vi "PicoReadPicoSingleBuffers.vi"(1 "enabled array":i16[](array[numeric]), 2 "Buffer and Transfer Settings":T3={"startIndex"=0, "Samples"=1000000, "Down Sample Ratio"=1, "Down-Sample Mode"=2147483648} {"Down-Sample Mode" items=["RAW none"=2147483648, "None"=0, "Aggregate"=1, "Decimate"=2, "Average"=4]; "Down Sample Ratio" step=1; "Samples" format="%_6p"}, 3 "Variant":string, 5 "Data Pointers":T2, 9 "Buffer Number":i32=1, 11 "error in (no error)":errorcluster) -> (6 "MaxBuffers (Max or non-aggregated)":T1, 8 "Min Buffers":T1, 15 "error out":errorcluster)   [LabVIEW 2010]
doc: "Read data from a single Picodata buffer."
uses:
  PicoBuffers.ctl
  Buffer and Transfer Settings.ctl
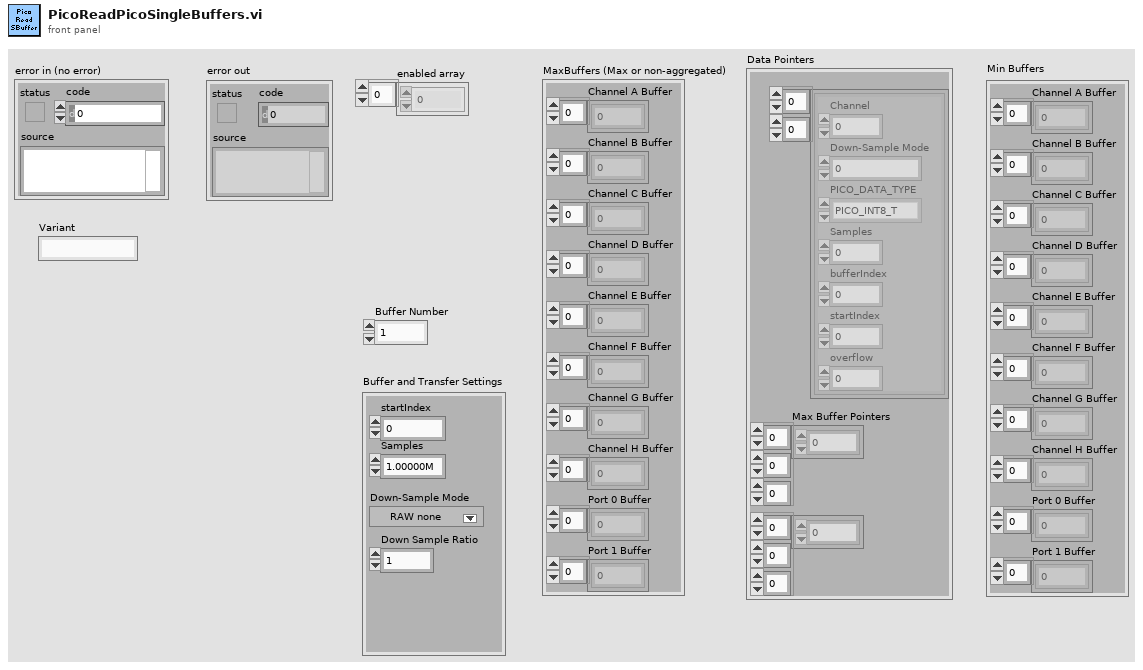
[diagram p1: front panel]
types:
  T1 = cluster{"Channel A Buffer":i16[], "Channel B Buffer":i16[], "Channel C Buffer":i16[], "Channel D Buffer":i16[], "Channel E Buffer":i16[], "Channel F Buffer":i16[], "Channel G Buffer":i16[], "Channel H Buffer":i16[], "Port 0 Buffer":i16[], "Port 1 Buffer":i16[]}
  T2 = typedef "PicoBuffers.ctl" = cluster{"Max Buffer Pointers":u64[][][], "Min Buffer Pointers":u64[][][], "StreamingDataInfo":cluster{"Channel":u32, "Down-Sample Mode":u32, "PICO_DATA_TYPE":enum32{"PICO_INT8_T", "PICO_INT16_T", "PICO_INT32_T", "PICO_UINT32_T", "PICO_INT64_T", ""}, "Samples":i32, "bufferIndex":u64, "startIndex":i32, "overflow":i16}[][]}
  T3 = typedef "Buffer and Transfer Settings.ctl" = cluster{"startIndex":u64, "Samples":u64, "Down Sample Ratio":u64, "Down-Sample Mode":u32}
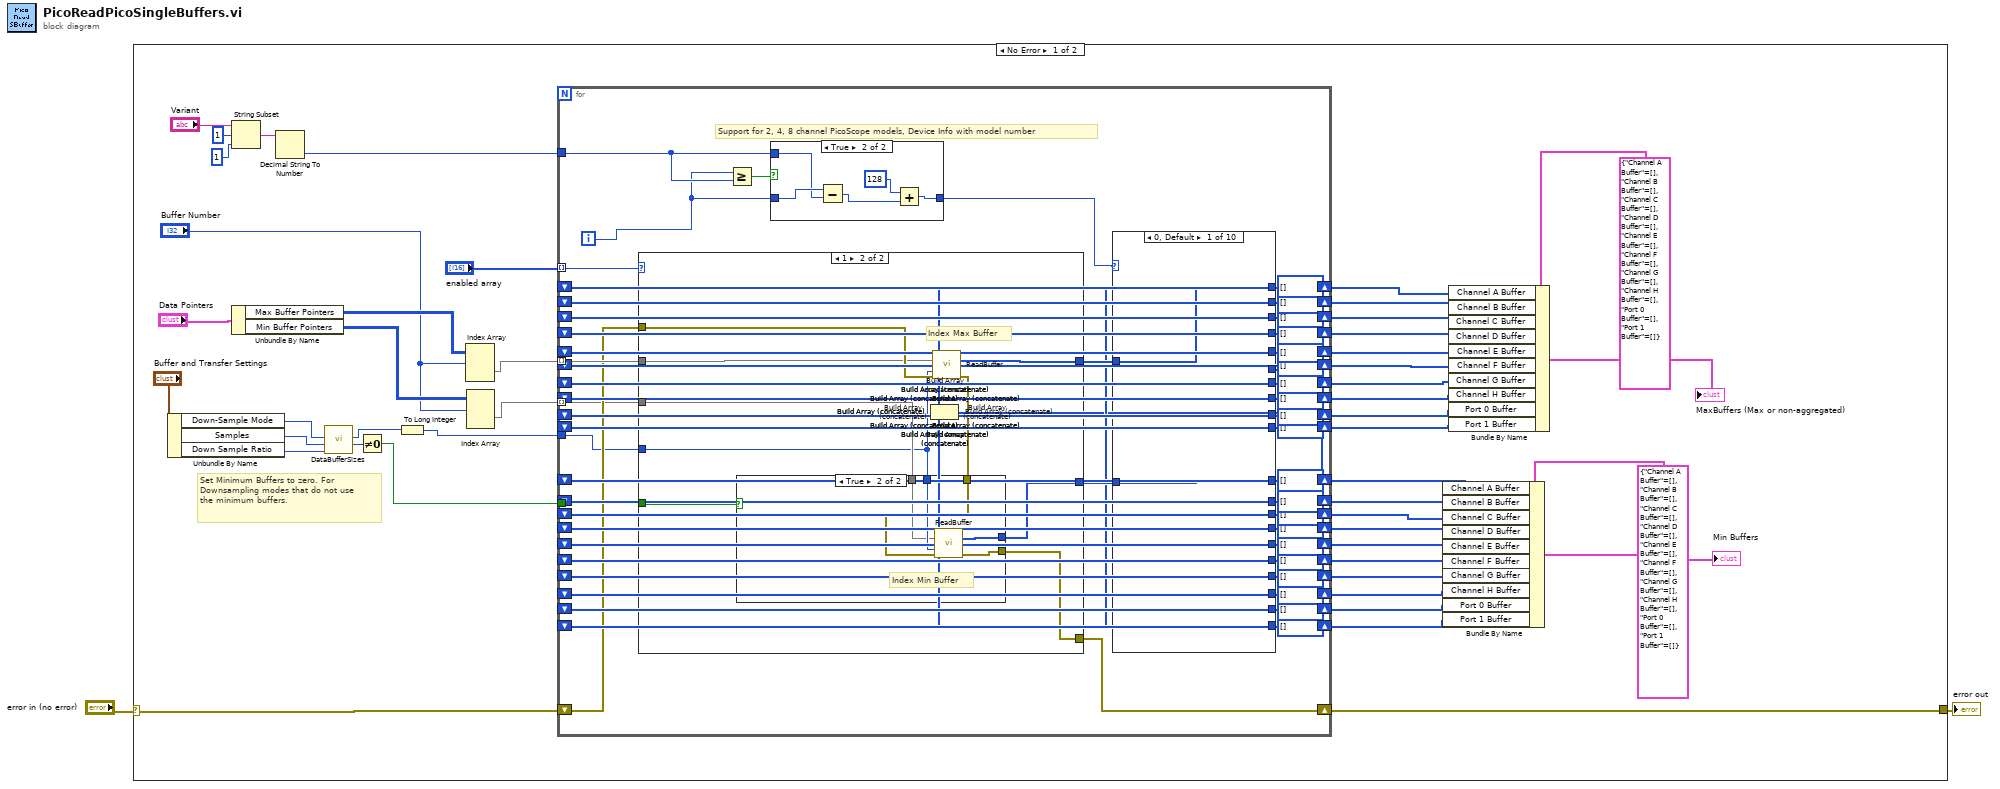
[diagram p0: block diagram]
diagram:
  n1 = case shown="No Error" "error in (no error)" {
    selector: "error in (no error)" -> [w66 w184]
    tunnel: [w68 w184] -> w1
    frame No Error {
      # "Set Minimum Buffers to zero. For Downsampling modes that do not use the minimum buffers."
      n2 = Unbundle By Name("Buffer and Transfer Settings") -> ("Down-Sample Mode"=w64:u32, "Samples"=w63:u64, "Down Sample Ratio"=w65:u64)
      n3 = Unbundle By Name("Data Pointers") -> ("Max Buffer Pointers"=w29:u64[][][], "Min Buffer Pointers"=w28:u64[][][])
      n4 = String Subset(string="Variant", offset (0)=1, length (rest)=1 ("length (rest)")) -> (substring=w57:string)
      n5 = Decimal String To Number(string=w57) -> (number=w23:i32)  [unwired: 2 in, 1 out]
      n6 = call "DataBufferSizes.vi"("Down Sample Ratio"=w65, "Number of Samples"=w63, "Down-Sample Mode"=w64) -> ("min Buffer Size"=w61:i32, "Max Buffer Size"=w59:i32)  [unwired: 7 in]
      n7 = Not Equal To 0?(x=w61) -> (x != 0?=w62:bool)
      n8 = To Long Integer(number=w59) -> (32bit integer=w60:i32)
      n9 = Index Array(array=w29, index (dim 0)="Buffer Number") -> (element=w27:u64[][])  [unwired: 2 in]
      n10 = Index Array(array=w28, index (dim 0)="Buffer Number") -> (element=w26:u64[][])  [unwired: 2 in]
      n11 = for {
        tunnel: "enabled array" -> [w140] mode=indexing
        tunnel: w27 -> [w141] mode=indexing
        shift-right: [w139] -> w68
        shift-left: w66 -> [w138]
        tunnel: w60 -> [w124]
        tunnel: w62 -> [w123]
        tunnel: w26 -> [w113] mode=indexing
        tunnel: w23 -> [w110]
        shift-right: [w107] -> w53
        shift-left: i16[] [] ("Output Array") -> [w108]
        shift-right: [w105] -> w52
        shift-left: i16[] [] ("Output Array") -> [w106]
        shift-right: [w103] -> w51
        shift-left: i16[] [] ("Output Array") -> [w104]
        shift-right: [w101] -> w50
        shift-left: i16[] [] ("Output Array") -> [w102]
        shift-right: [w99] -> w49
        shift-left: i16[] [] ("Output Array") -> [w100]
        shift-right: [w97] -> w48
        shift-left: i16[] [] ("Output Array") -> [w98]
        shift-right: [w95] -> w42
        shift-left: i16[] [] ("Output Array") -> [w96]
        shift-right: [w93] -> w47
        shift-left: i16[] [] ("Output Array") -> [w94]
        shift-right: [w91] -> w46
        shift-left: i16[] [] ("Output Array") -> [w92]
        shift-right: [w89] -> w45
        shift-left: i16[] [] ("Output Array") -> [w90]
        shift-right: [w87] -> w44
        shift-left: i16[] [] ("Output Array") -> [w88]
        shift-right: [w85] -> w43
        shift-left: i16[] [] ("Output Array") -> [w86]
        shift-right: [w83] -> w39
        shift-left: i16[] [] ("Output Array") -> [w84]
        shift-right: [w81] -> w38
        shift-left: i16[] [] ("Output Array") -> [w82]
        shift-right: [w79] -> w37
        shift-left: i16[] [] ("Output Array") -> [w80]
        shift-right: [w77] -> w36
        shift-left: i16[] [] ("Output Array") -> [w78]
        shift-right: [w75] -> w35
        shift-left: i16[] [] ("Output Array") -> [w76]
        shift-right: [w73] -> w34
        shift-left: i16[] [] ("Output Array") -> [w74]
        shift-right: [w71] -> w33
        shift-left: i16[] [] ("Output Array") -> [w72]
        shift-right: [w69] -> w32
        shift-left: i16[] [] ("Output Array") -> [w70]
        i -> [w109]
        # "Support for 2, 4, 8 channel PicoScope models, Device Info with model number"
        n12 = case shown="1" w140 {
          tunnel: w141 -> [_ w171]
          tunnel: [_ w177] -> w137
          tunnel: [_ w176] -> w136
          tunnel: w138 -> [w168 w175]
          tunnel: [w168 w173] -> w139
          tunnel: w124 -> [_ w169]
          tunnel: w123 -> [_ w172]
          tunnel: w113 -> [_ w170]
          frame 0, Default {
          }
          frame 1 {
            # "Index Max Buffer"
            n13 = call "ReadBuffer.vi"("Pointer and BufferSize"=w171, "Buffer size"=w169, "error in (no error)"=w175) -> ("Output Array"=w177:i16[], "error out"=w174:errorcluster)  [unwired: 11 in]
            n14 = case shown="True" w172 {
              tunnel: [_ w183] -> w176
              tunnel: w174 -> [w178 w182]
              tunnel: [w178 w181] -> w173
              tunnel: w169 -> [_ w180]
              tunnel: w170 -> [_ w179]
              frame False {
              }
              frame True {
                # "Index Min Buffer"
                n15 = call "ReadBuffer.vi"("Pointer and BufferSize"=w179, "Buffer size"=w180, "error in (no error)"=w182) -> ("Output Array"=w183:i16[], "error out"=w181:errorcluster)  [unwired: 11 in]
              }
            }
          }
        }
        n16 = Greater Or Equal?(x=w109, y=w110) -> (x >= y?=w112:bool)
        n17 = case shown="True" w112 {
          tunnel: w109 -> [w142 w144]
          tunnel: [w142 w146] -> w111
          tunnel: w110 -> [_ w143]
          frame False {
          }
          frame True {
            n18 = Subtract(x=w144, y=w143) -> (x-y=w145:i32)
            n19 = Add(x=128, y=w145) -> (x+y=w146:i32)
          }
        }
        n20 = case shown="0, Default" w111 {
          tunnel: w137 -> [w149 w151 w153 w155 w157 w159 w161 w163 w165 w167]
          tunnel: [w149 _ _ _ _ _ _ _ _ _] -> w122
          tunnel: [_ w151 _ _ _ _ _ _ _ _] -> w129
          tunnel: [_ _ w153 _ _ _ _ _ _ _] -> w128
          tunnel: [_ _ _ w155 _ _ _ _ _ _] -> w127
          tunnel: [_ _ _ _ w157 _ _ _ _ _] -> w126
          tunnel: [_ _ _ _ _ w159 _ _ _ _] -> w125
          tunnel: w136 -> [w148 w150 w152 w154 w156 w158 w160 w162 w164 w166]
          tunnel: [w148 _ _ _ _ _ _ _ _ _] -> w135
          tunnel: [_ w150 _ _ _ _ _ _ _ _] -> w134
          tunnel: [_ _ w152 _ _ _ _ _ _ _] -> w133
          tunnel: [_ _ _ w154 _ _ _ _ _ _] -> w132
          tunnel: [_ _ _ _ w156 _ _ _ _ _] -> w131
          tunnel: [_ _ _ _ _ w158 _ _ _ _] -> w130
          tunnel: [_ _ _ _ _ _ w161 _ _ _] -> w121
          tunnel: [_ _ _ _ _ _ w160 _ _ _] -> w120
          tunnel: [_ _ _ _ _ _ _ w163 _ _] -> w119
          tunnel: [_ _ _ _ _ _ _ w162 _ _] -> w118
          tunnel: [_ _ _ _ _ _ _ _ w165 _] -> w117
          tunnel: [_ _ _ _ _ _ _ _ w164 _] -> w116
          tunnel: [_ _ _ _ _ _ _ _ _ w167] -> w115
          tunnel: [_ _ _ _ _ _ _ _ _ w166] -> w114
          frame 0, Default {
          }
          frame 1 {
          }
          frame 2 {
          }
          frame 3 {
          }
          frame 4 {
          }
          frame 5 {
          }
          frame 6 {
          }
          frame 7 {
          }
          frame 128 {
          }
          frame 129 {
          }
        }
        n21 = Build Array (concatenate)(w70, w114) -> (w69:i16[])
        n22 = Build Array (concatenate)(w72, w115) -> (w71:i16[])
        n23 = Build Array (concatenate)(w74, w116) -> (w73:i16[])
        n24 = Build Array (concatenate)(w76, w117) -> (w75:i16[])
        n25 = Build Array (concatenate)(w78, w118) -> (w77:i16[])
        n26 = Build Array (concatenate)(w80, w119) -> (w79:i16[])
        n27 = Build Array (concatenate)(w82, w120) -> (w81:i16[])
        n28 = Build Array (concatenate)(w84, w121) -> (w83:i16[])
        n29 = Build Array (concatenate)(w86, w125) -> (w85:i16[])
        n30 = Build Array (concatenate)(w88, w126) -> (w87:i16[])
        n31 = Build Array (concatenate)(w90, w127) -> (w89:i16[])
        n32 = Build Array (concatenate)(w92, w128) -> (w91:i16[])
        n33 = Build Array (concatenate)(w94, w129) -> (w93:i16[])
        n34 = Build Array (concatenate)(w96, w122) -> (w95:i16[])
        n35 = Build Array (concatenate)(w98, w130) -> (w97:i16[])
        n36 = Build Array (concatenate)(w100, w131) -> (w99:i16[])
        n37 = Build Array (concatenate)(w102, w132) -> (w101:i16[])
        n38 = Build Array (concatenate)(w104, w133) -> (w103:i16[])
        n39 = Build Array (concatenate)(w106, w134) -> (w105:i16[])
        n40 = Build Array (concatenate)(w108, w135) -> (w107:i16[])
      }
      n41 = Bundle By Name(cluster=T1 {"Channel A Buffer"=[], "Channel B Buffer"=[], "Channel C Buffer"=[], "Channel D Buffer"=[], "Channel E Buffer"=[], "Channel F Buffer"=[], "Channel G Buffer"=[], "Channel H Buffer"=[], "Port 0 Buffer"=[], "Port 1 Buffer"=[]} ("input cluster"), "Channel A Buffer"=w53, "Channel B Buffer"=w52, "Channel C Buffer"=w51, "Channel D Buffer"=w50, "Channel E Buffer"=w49, "Channel F Buffer"=w48, "Channel G Buffer"=w38, "Channel H Buffer"=w36, "Port 0 Buffer"=w34, "Port 1 Buffer"=w32) -> (→"Min Buffers":T1)
      n42 = Bundle By Name(cluster=T1 {"Channel A Buffer"=[], "Channel B Buffer"=[], "Channel C Buffer"=[], "Channel D Buffer"=[], "Channel E Buffer"=[], "Channel F Buffer"=[], "Channel G Buffer"=[], "Channel H Buffer"=[], "Port 0 Buffer"=[], "Port 1 Buffer"=[]} ("input cluster"), "Channel A Buffer"=w42, "Channel B Buffer"=w47, "Channel C Buffer"=w46, "Channel D Buffer"=w45, "Channel E Buffer"=w44, "Channel F Buffer"=w43, "Channel G Buffer"=w39, "Channel H Buffer"=w37, "Port 0 Buffer"=w35, "Port 1 Buffer"=w33) -> (→"MaxBuffers (Max or non-aggregated)":T1)
    }
    frame Error {
    }
  }
  "error out" <- w1
